vi "assembly sort.vi"(8 "Right Read MIN":i32=5, 9 "Signal Tag A":string[](array[string]), 10 "連続排除配列":string, 11 "Signal Profile Table A":string[][](table) caption="Singla Profile Table") -> (0 "assembly C":T1, 1 "Selected S IDX":i32[](array[numeric]), 2 "Selected S Filename":string[](array[string]), 3 "Long Assembly":bool[][](array[boolean]), 5 "Signal#":i32)   [LabVIEW 2018]
panel:
  out "S IDX":string[](array[string])
  out "Signal Tag A 2":string[](array[string])
  out "サイズ 2":i32
  out "サイズ":i32[](array[numeric])
  out "Assembly ratio":dbl
  out "Long Signal#":i32
  out "Seq SN":i32
  out "Seq EN":i32
  out "File name":string[](array[string])
  out "Direction":string[](array[string])
  out "Seq EN":string[](array[string])
  out "Mx Right No":string[](array[string])
  out "Seq SNo":string[](array[string])
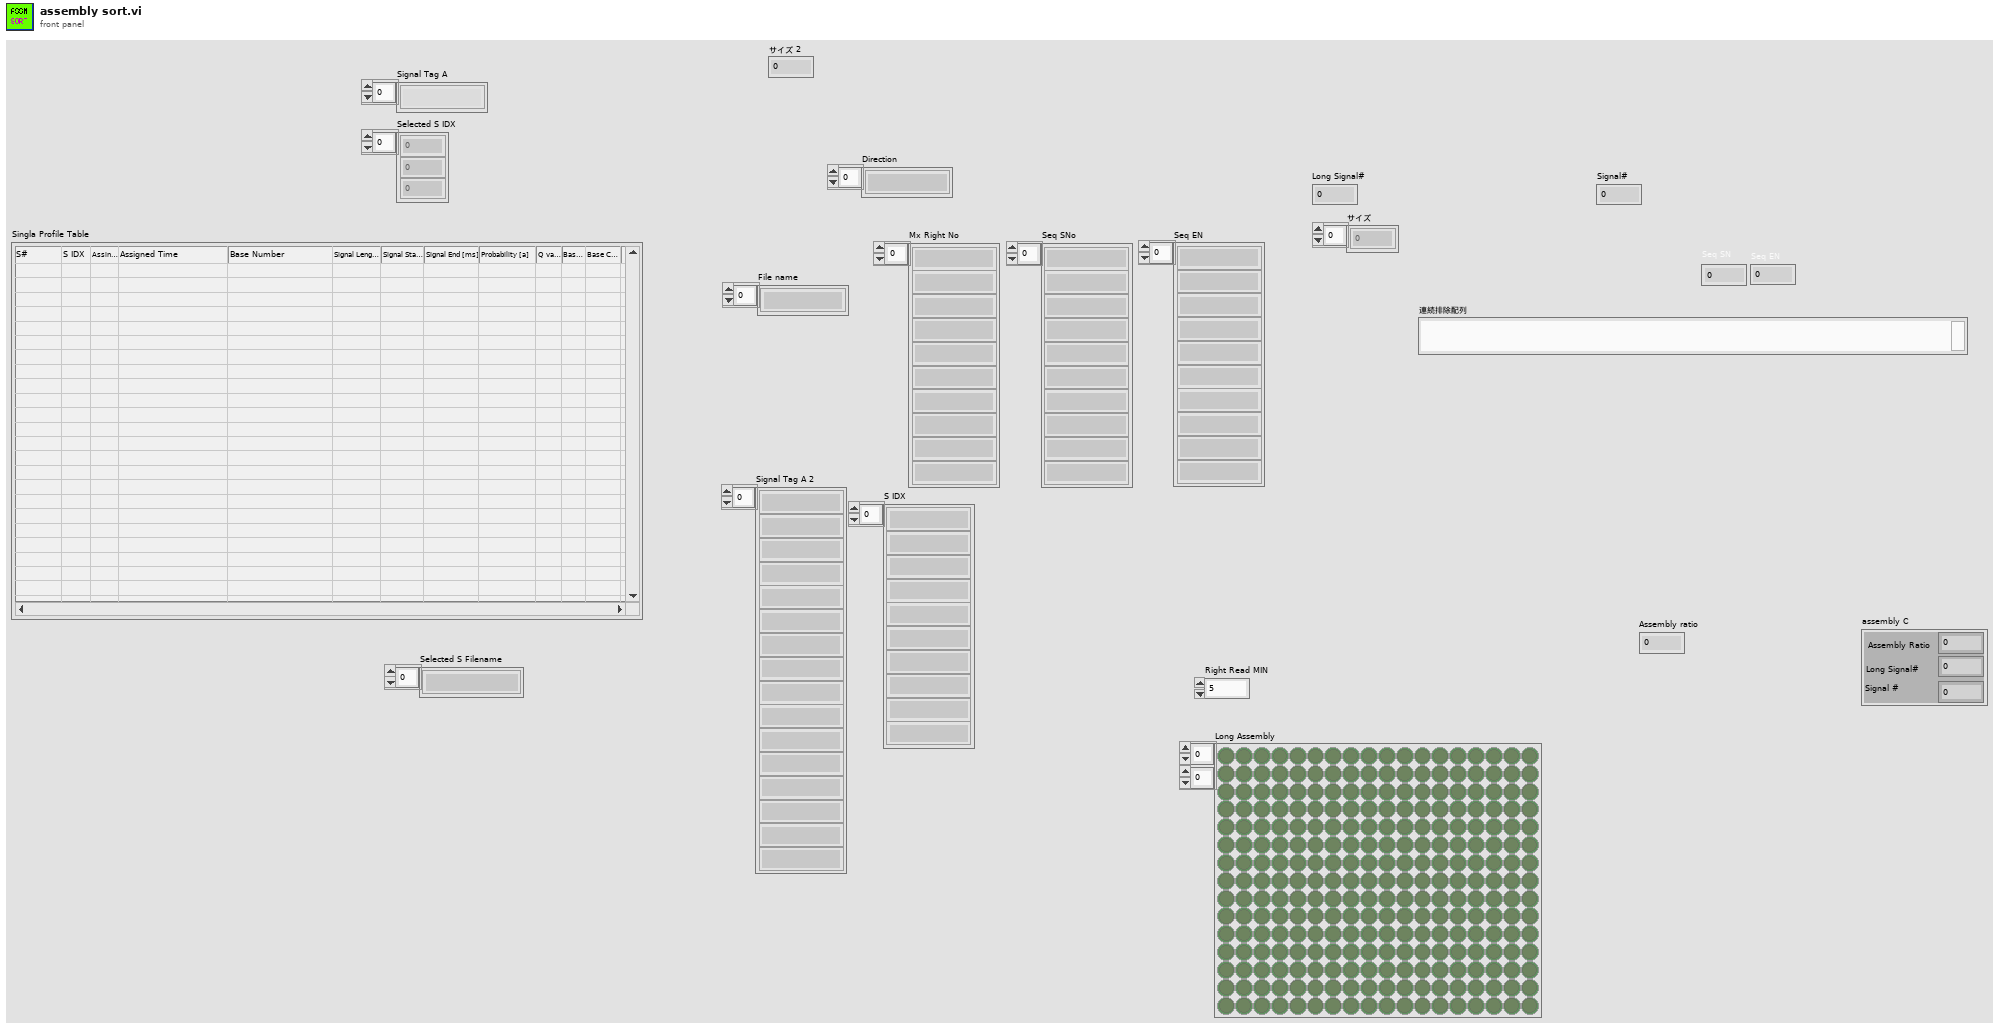
[diagram p1: front panel]
types:
  T1 = cluster{"Assembly Ratio":dbl, "Long Signal#":i32, "Signal #":i32}
  T2 = cluster{i32, "offset past number":i32, i32, string, string, string}[]
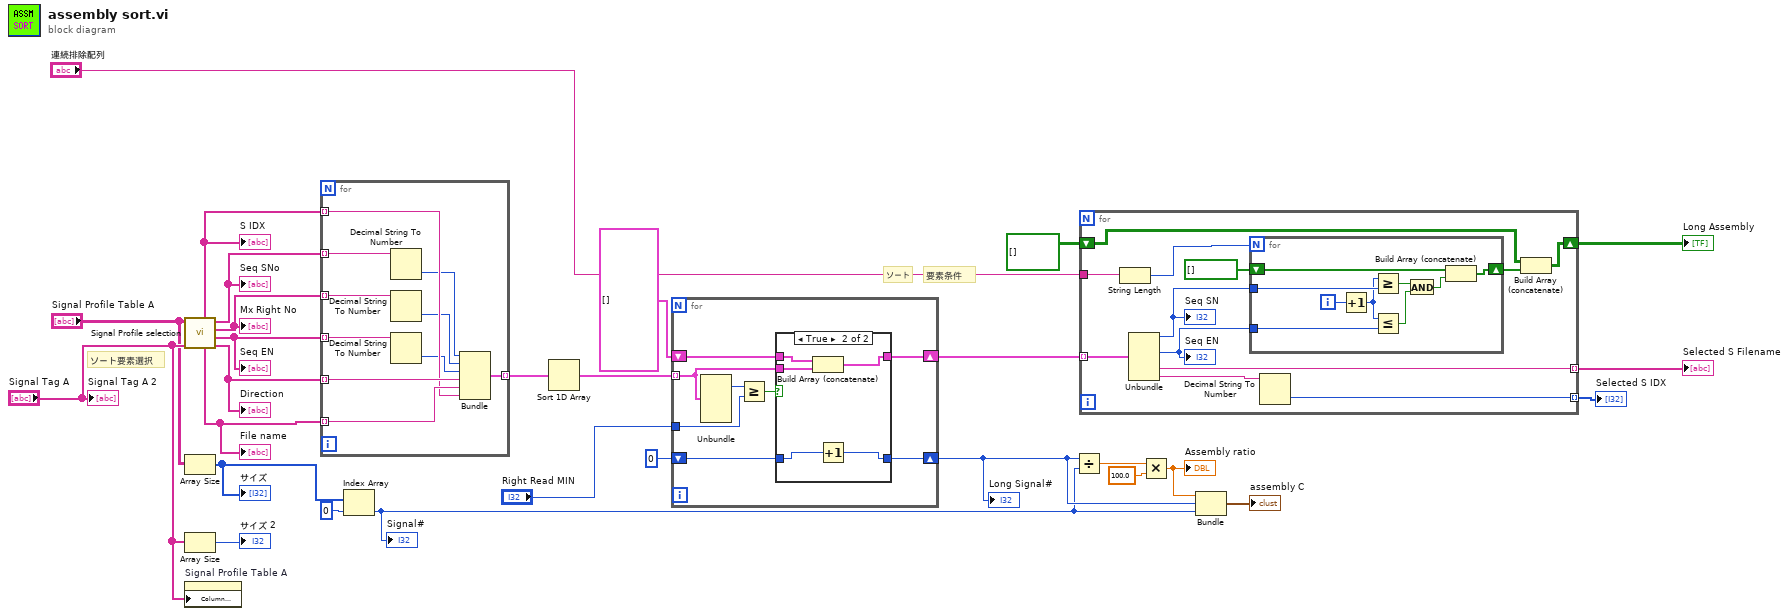
[diagram p0: block diagram]
diagram:
  # "要素条件"
  # "ソート"
  # "ソート要素選択"
  n1 = call "Signal Profile selection.vi"("Signal Tag A"="Signal Tag A", "Signal Profile Table A"="Signal Profile Table A") -> ("Direction"=w3:string[], "Seq ENo"=w4:string[], "Mx Right No"=w5:string[], "Seq SNo"=w6:string[], "File name"=w7:string[], "S IDX"=w2:string[])  [unwired: 3 in, 1 out]
  "Seq SNo" <- w6
  "Mx Right No" <- w5
  "Seq EN" <- w4
  "Direction" <- w3
  "File name" <- w7
  "S IDX" <- w2
  n2 = Array Size(array="Signal Profile Table A") -> (size(s)=w16:i32[])
  "サイズ" <- w16
  n3 = Array Size(array="Signal Tag A") -> (size(s)=→"サイズ 2":i32)
  n4 = property on="Signal Profile Table A" class="Tbl (strict)"("Column Headers[]"="Signal Tag A") -> ()  [unwired: 2 in, 2 out]
  n5 = for {
    tunnel: [w38] -> w28 mode=indexing
    tunnel: w6 -> [w34] mode=indexing
    tunnel: w5 -> [w30] mode=indexing
    tunnel: w4 -> [w32] mode=indexing
    tunnel: w3 -> [w37] mode=indexing
    tunnel: w7 -> [w36] mode=indexing
    tunnel: w2 -> [w35] mode=indexing
    n6 = Decimal String To Number(string=w34) -> (number=w33:i32)  [unwired: 2 in, 1 out]
    n7 = Decimal String To Number(string=w30) -> (number=w29:i32)  [unwired: 2 in, 1 out]
    n8 = Decimal String To Number(string=w32) -> (number=w31:i32)  [unwired: 2 in, 1 out]
    n9 = Bundle(w33, w29, w31, w37, w36, w35) -> (w38:cluster{i32, i32, i32, string, string, string})  [unwired: 1 in]
  }
  n10 = Index Array(array=w16, index=0 ("指標")) -> (element=w14:i32)
  "Signal#" <- w14
  n11 = Sort 1D Array(array=w28) -> (sorted array=w26:cluster{i32, i32, i32, string, string, string}[])
  n12 = for {
    tunnel: w26 -> [w46] mode=indexing
    shift-right: [w45] -> w13
    shift-left: T2 [] -> [w44]
    tunnel: "Right Read MIN" -> [w42]
    shift-right: [w40] -> w17
    shift-left: 0 -> [w41]
    n13 = Unbundle(w46) -> (w39:i32)  [unwired: 5 out]
    n14 = Greater Or Equal?(x=w39, y=w42) -> (x >= y?=w43:bool)
    n15 = case shown="True" w43 {
      tunnel: w46 -> [_ w53]
      tunnel: [w48 w52] -> w45
      tunnel: w44 -> [w48 w51]
      tunnel: w41 -> [w47 w50]
      tunnel: [w47 w49] -> w40
      frame False {
      }
      frame True {
        n16 = Build Array (concatenate)(w51, w53) -> (w52:T2)
        n17 = Increment(x=w50) -> (x+1=w49:i32)
      }
    }
  }
  "Long Signal#" <- w17
  n18 = Divide(x=w17, y=w14) -> (x/y=w21:dbl)
  n19 = for {
    tunnel: w13 -> [w65] mode=indexing
    tunnel: "連続排除配列" -> [w64]
    shift-right: [w60] -> w24
    shift-left: bool[][] [] -> [w59]
    tunnel: [w57] -> w12 mode=indexing
    tunnel: [w56] -> w11 mode=indexing
    n20 = String Length(string=w64) -> (length=w63:i32)
    n21 = Unbundle(w65) -> (w55:i32, w54:i32, w56:string, w58:string)  [unwired: 2 out]
    "Seq SN" <- w55
    "Seq EN" <- w54
    n22 = for {
      N: w63 -> [_]
      tunnel: w55 -> [w67]
      tunnel: w54 -> [w69]
      shift-right: [w74] -> w61
      shift-left: bool[] [] -> [w73]
      i -> [w68]
      n23 = Increment(x=w68) -> (x+1=w66:i32)
      n24 = Greater Or Equal?(x=w66, y=w67) -> (x >= y?=w72:bool)
      n25 = Less Or Equal?(x=w66, y=w69) -> (x <= y?=w70:bool)
      n26 = And(x=w72, y=w70) -> (x .and. y?=w71:bool)
      n27 = Build Array (concatenate)(w73, w71) -> (w74:bool[])
    }
    n28 = Decimal String To Number(string=w58) -> (number=w57:i32)  [unwired: 2 in, 1 out]
    n29 = Build Array (concatenate)(w59, w61) -> (w60:bool[][])
  }
  "Long Assembly" <- w24
  "Selected S IDX" <- w12
  "Selected S Filename" <- w11
  n30 = Multiply(x=w21, y=100.0) -> (x*y=w19:dbl)
  "Assembly ratio" <- w19
  n31 = Bundle(w19, w17, w14) -> (→"assembly C":cluster{dbl, i32, i32})  [unwired: 1 in]
  "Signal Tag A 2" <- "Signal Tag A"
